vi "libssh2_session_method_pref.vi"(8 "error in (no error)":errorcluster, 9 "prefs":string, 10 "method_type":T1, 11 "session":T2) -> (0 "error out":errorcluster)   [LabVIEW 2017, in "libssh2.lvlib"]
doc: "Set the preferred methods to negotiate for a session."
uses:
  libssh2.lvlib
  Session Refnum.ctl
  libssh2_method_type.ctl
  Not A Session.vi
  <vilib>/Utility/error.llb/Error Cluster From Error Code.vi
  Global Settings.vi
  Read Session Refnum.vi
  <vilib>/Utility/semaphor.llb/Acquire Semaphore.vi
  <vilib>/Utility/semaphor.llb/Release Semaphore.vi
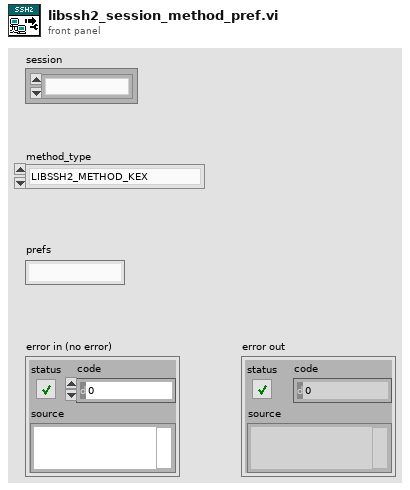
[diagram p1: front panel]
types:
  T1 = typedef "libssh2.lvlib/libssh2_method_type.ctl" = enum16{"LIBSSH2_METHOD_KEX", "LIBSSH2_METHOD_HOSTKEY", "LIBSSH2_METHOD_CRYPT_CS", "LIBSSH2_METHOD_CRYPT_SC", "LIBSSH2_METHOD_MAC_CS", "LIBSSH2_METHOD_MAC_SC", "LIBSSH2_METHOD_COMP_CS", "LIBSSH2_METHOD_COMP_SC", "LIBSSH2_METHOD_LANG_CS", "LIBSSH2_METHOD_LANG_SC", "LIBSSH2_METHOD_SIGN_ALGO"}
  T2 = typedef "libssh2.lvlib/Session Refnum.ctl" = refnum<k1>
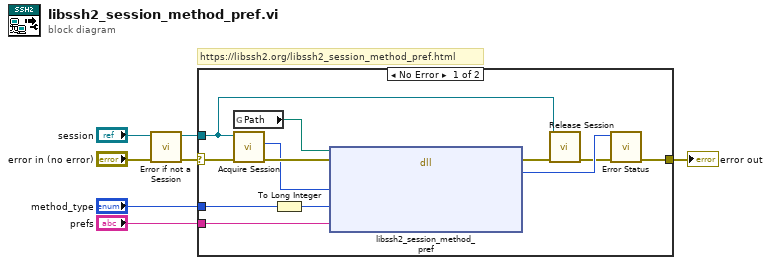
[diagram p0: block diagram]
diagram:
  # "https://libssh2.org/libssh2_session_method_pref.html"
  n1 = call "Error if not a Session.vi"("error in (no error)"="error in (no error)", "session"="session") -> ("error out"=w5:errorcluster, "session out"=w3:T2)  [unwired: 8 in]
  n2 = case shown="No Error" w5 {
    selector: w5 -> [w18 w20]
    tunnel: [w12 w20] -> w7
    tunnel: w3 -> [w8 _]
    tunnel: "method_type" -> [w14 _]
    tunnel: "prefs" -> [w10 _]
    frame No Error {
      n3 = global read "Global Settings.vi" "Path"() -> (w15:path)
      n4 = call "Acquire Session.vi"("error in (no error)"=w18, "session"=w8) -> ("error out"=w17:errorcluster, "LIBSSH2_SESSION*"=w16:u64)  [unwired: 7 in, 1 out]
      n5 = To Long Integer(number=w14) -> (32bit integer=w13:i32)
      n6 = dll-call lib="?" fn="libssh2_session_method_pref"(path in=w15, error in=w17, "session"=w16, "method_type"=w13, "prefs"=w10) -> (error out=w19:errorcluster, "return value"=w11:i32)  [unwired: 4 in, 1 out]
      n7 = call "Release Session.vi"("error in (no error)"=w19, "session"=w8) -> ("error out"=w9:errorcluster)  [unwired: 9 in]
      n8 = call "Error Status.vi"("error in (no error)"=w9, "return value"=w11) -> ("error out"=w12:errorcluster)  [unwired: 8 in, 1 out]
    }
    frame Error {
    }
  }
  "error out" <- w7
